vi "Get ECAT Variable Contents.vi"(8 "error in (no error)":errorcluster, 11 "ECAT Variablenobjekt in":refnum<k21>[](array[refnum])) -> (0 "error out":errorcluster, 2 "All Variables Contents":T1[](array[typedef]), 3 "ECAT Variablenobjekt out":refnum<k21>[](array[refnum]))   [LabVIEW 2020, in "SEECD System Explorer.lvlib"]
uses:
  SEECD System Explorer.lvlib
  Type Defs/IOV Container Contents.ctl
  <resource>/objmgr/ni.var.rc
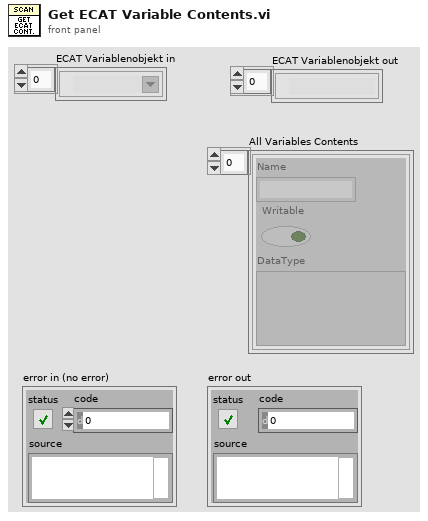
[diagram p1: front panel]
types:
  T1 = typedef "SEECD System Explorer.lvlib/IOV Container Contents.ctl" = cluster{"Name":string, "Writable":bool, "DataType":variant}
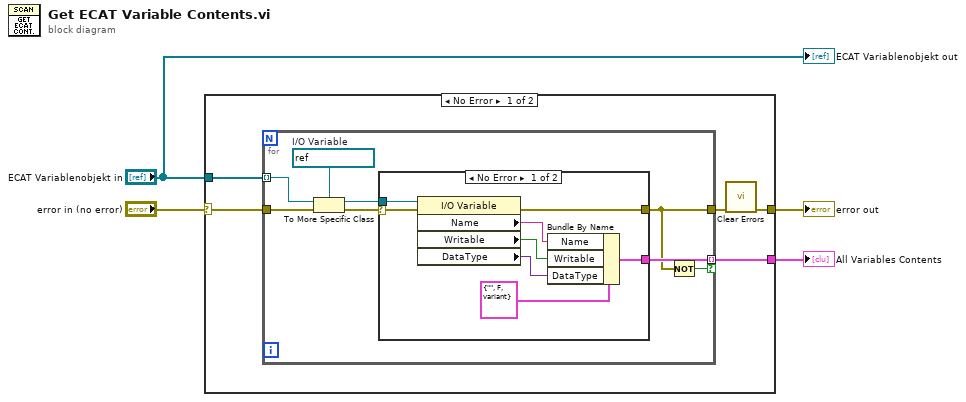
[diagram p0: block diagram]
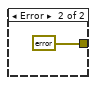
[diagram p2: hidden frame]
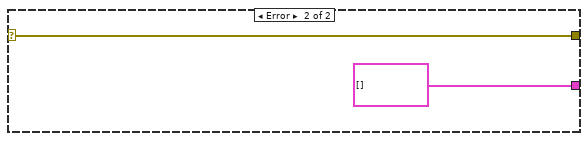
[diagram p3: hidden frame]
diagram:
  n1 = case shown="No Error" "error in (no error)" {
    selector: "error in (no error)" -> [w7 w28]
    tunnel: [w5 w28] -> w4
    tunnel: [w8 T1[] []] -> w3
    tunnel: "ECAT Variablenobjekt in" -> [w6 _]
    frame No Error {
      n2 = for {
        tunnel: w6 -> [w14] mode=indexing
        tunnel: [w17] -> w8 mode=indexing if=w10
        tunnel: w7 -> [w15]
        tunnel: [w11] -> w9
        w16 = refnum<k21> refnum  # I/O Variable
        n3 = To More Specific Class(target class=w16, reference=w14, error in=w15) -> (specific class reference=w13:refnum<k21>, error out=w12:errorcluster)
        n4 = case shown="No Error" w12 {
          selector: w12 -> [w18 _]
          tunnel: [w25 errorcluster {"status"=FALSE, "code"=0, "source"=""} ("error out")] -> w11
          tunnel: [w20 _] -> w17
          tunnel: w13 -> [w19 _]
          frame No Error {
            n5 = property class="I/O Variable"(reference=w19, error in=w18) -> (error out=w25:errorcluster, "Name"=w23:string, "Writable"=w22:bool, "DataType"=w21:variant)  [unwired: 1 out]
            n6 = Bundle By Name(cluster=T1 {"Name"="", "Writable"=FALSE, "DataType"=variant} ("IO Variable Container Contents"), "Name"=w23, "Writable"=w22, "DataType"=w21) -> (w20:T1)
          }
          frame Error {
          }
        }
        n7 = Not(x=w11) -> (.not. x?=w10:bool)
      }
      n8 = call <vilib>:"Clear Errors.vi"("error in (no error)"=w9) -> ("error out"=w5:errorcluster)  [unwired: 5 in, 1 out]
    }
    frame Error {
    }
  }
  "error out" <- w4
  "All Variables Contents" <- w3
  "ECAT Variablenobjekt out" <- "ECAT Variablenobjekt in"
